vi "destroy point buffer.vi"(11 "point buffer":refnum<data-value>) -> (0 "error out":errorcluster)   [LabVIEW 2020, in "nominal core steps.lvlib"]
doc: "Immediately destroy the point buffer. Does not flush."
uses:
  nominal core steps.lvlib
  points buffer.ctl
  single point.ctl
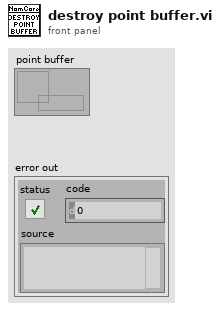
[diagram p1: front panel]
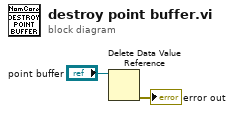
[diagram p0: block diagram]
diagram:
  n1 = Delete Data Value Reference(data value reference="point buffer") -> (error out=→"error out":errorcluster)  [unwired: 1 in, 1 out]
